vi "FlyWheelSim_Example.vi"() -> ()   [LabVIEW 2019]
uses:
  <vilib>/Rock Robotics/WPI/ThirdParty/JAS_Junk/TrajLib/TypeDef/DCMOTOR.CTL
  <vilib>/Rock Robotics/WPI/ThirdParty/JAS_Junk/TrajLib/TypeDef/LINEAR_SYSTEM.ctl
  <vilib>/Analysis/Matrix/Datatypes/RealMatrix.ctl
  <vilib>/Rock Robotics/WPI/ThirdParty/JAS_Junk/TrajLib/TypeDef/LINEAR_QUADRATIC_REGULATOR.ctl
  <vilib>/Rock Robotics/WPI/ThirdParty/JAS_Junk/TrajLib/TypeDef/KALMAN_FILTER.ctl
  <vilib>/Rock Robotics/WPI/ThirdParty/JAS_Junk/TrajLib/TypeDef/LINEAR_SYSTEM_LOOP.ctl
  <vilib>/Rock Robotics/WPI/ThirdParty/JAS_Junk/TrajLib/TypeDef/LINEAR_PLANT_INV_FF.ctl
  <vilib>/Rock Robotics/WPI/ThirdParty/JAS_Junk/TrajLib/TypeDef/FLYWHEEL_SIM.ctl
  <vilib>/Rock Robotics/WPI/ThirdParty/JAS_Junk/TrajLib/TypeDef/LINEAR_SYSTEM_SIM.ctl
  <vilib>/Rock Robotics/WPI/ThirdParty/JAS_Junk/TrajLib/MatBuilder_Create.vi
  <vilib>/Rock Robotics/WPI/ThirdParty/JAS_Junk/TrajLib/LinearFilter_ResetToValue.vi
  <vilib>/Rock Robotics/WPI/ThirdParty/JAS_Junk/TrajLib/LinearFilter_Calculate.vi
  <vilib>/Rock Robotics/WPI/ThirdParty/JAS_Junk/TrajLib/LinearFilter_MovingAverage.vi
  <vilib>/Rock Robotics/WPI/ThirdParty/JAS_Junk/TrajLib/LinearFilter_LowPassBW1.vi
  <vilib>/Rock Robotics/WPI/ThirdParty/JAS_Junk/TrajLib/LinearFilter_LowPassBW2.vi
  <vilib>/Rock Robotics/WPI/ThirdParty/JAS_Junk/TrajLib/LinearFilter_HighPassBW1.vi
  <vilib>/Rock Robotics/WPI/ThirdParty/JAS_Junk/TrajLib/LinearFilter_HighPassBW2.vi
  <vilib>/Rock Robotics/WPI/ThirdParty/JAS_Junk/TrajLib/Trajectory_Library.lvlib
  <vilib>/Analysis/Matrix/NI_Matrix.lvlib
panel:
  in  "Tab Control":T1(tab)
  out "Motor Current":dbl format="%20.3f"
  out "Battery \nVoltage":dbl format="%20.3f"
  in  "Shoot ball":bool
  out "CO Chart":T2(graph)
  in  "Shooter On/Off":bool
  out "Encoer Speed\nRad/Sec":dbl(slide) scale=0.0..300.0
  out "Speed":dbl format="%20.3f"
  out "Kalman Filtered\nSpeed":dbl format="%20.3f"
  out "PV Chart":T3(graph)
  out "Error":bool
  out "Motor Volt Dmd (CO)":dbl format="%20.3f"
  out "shoot Start":bool
  out "Shoot Done":bool
  out "Shooter Motor":T4 {"Jr_KgM2" format="%13.5p"; "L_H" format="%13.5p"; "Kt_NMPerAmp" format="%13.5p"; "KvINV_RadPerSecPerVolt" format="%13.5p"; "R_Ohms" format="%13.5p"; "FreeSpeed_RadPerSec" format="%13.5p"; "FreeCurrent_Amps" format="%13.5p"; "StallCurrent_Amps" format="%13.5p"; "StallTorque_NM" format="%13.5p"; "nominalVoltage_Volts" format="%13.5p"}
  out "m_flywheelPlant":T5
  out "m_FlyWheelSim":T7 {"GearBox"."Jr_KgM2" format="%13.5p"; "GearBox"."L_H" format="%13.5p"; "GearBox"."Kt_NMPerAmp" format="%13.5p"; "GearBox"."KvINV_RadPerSecPerVolt" format="%13.5p"; "GearBox"."R_Ohms" format="%13.5p"; "GearBox"."FreeSpeed_RadPerSec" format="%13.5p"; "GearBox"."FreeCurrent_Amps" format="%13.5p"; "GearBox"."StallCurrent_Amps" format="%13.5p"; "GearBox"."StallTorque_NM" format="%13.5p"; "GearBox"."nominalVoltage_Volts" format="%13.5p"}
  out "Shooting A":T6
  out "Shooting B":T6
  out "KalmanFilter":T9
  out "Kalman Error":errorcluster
  out "LinearQuadraticRegulator":T10
  out "LQR Error":bool
  out "Linear System Loop":T11
  out "LinSysLoop_Error":bool
  # "<States,States>"
  # "<States,Inputs>"
  # "<Outputs,States>"
  # "<Outputs,Inputs>"
  # "<States, 1>"
  # "<Outputs, 1>"
  # "<Inputs, 1>"
  # "<Outputs, 1>"
  # "<States,States>"
  # "<States,Inputs>"
  # "<Outputs,States>"
  # "<Outputs,Inputs>"
  # "Steady State Gain  \n<States,Outputs>"
  # "State Estimate <Statess,1>"
  # "<States,States>"
  # "<States,Inputs>"
  # "<Outputs,States>"
  # "<Outputs,Inputs>"
  # "Ref State <States,1>"
  # "Comp and capped \noutput <Inputs,1>"
  # "Controller gain\n<Inputs,States>"
  # "<States,1>"
  # "<FUTURE --- CLAMP TYPE -- For now\nuse Normalize>"
  # "Steady State Gain  \n<States,Outputs>"
  # "State Estimate <Statess,1>"
  # "<States,States>"
  # "<States,Inputs>"
  # "<Outputs,States>"
  # "<Outputs,Inputs>"
  # "<States,1>"
  # "<Inputs,1>"
  # "<States,Inputs>"
  # "<States,States>"
  # "Ref State <States,1>"
  # "Comp and capped \noutput <Inputs,1>"
  # "Controller gain\n<Inputs,States>"
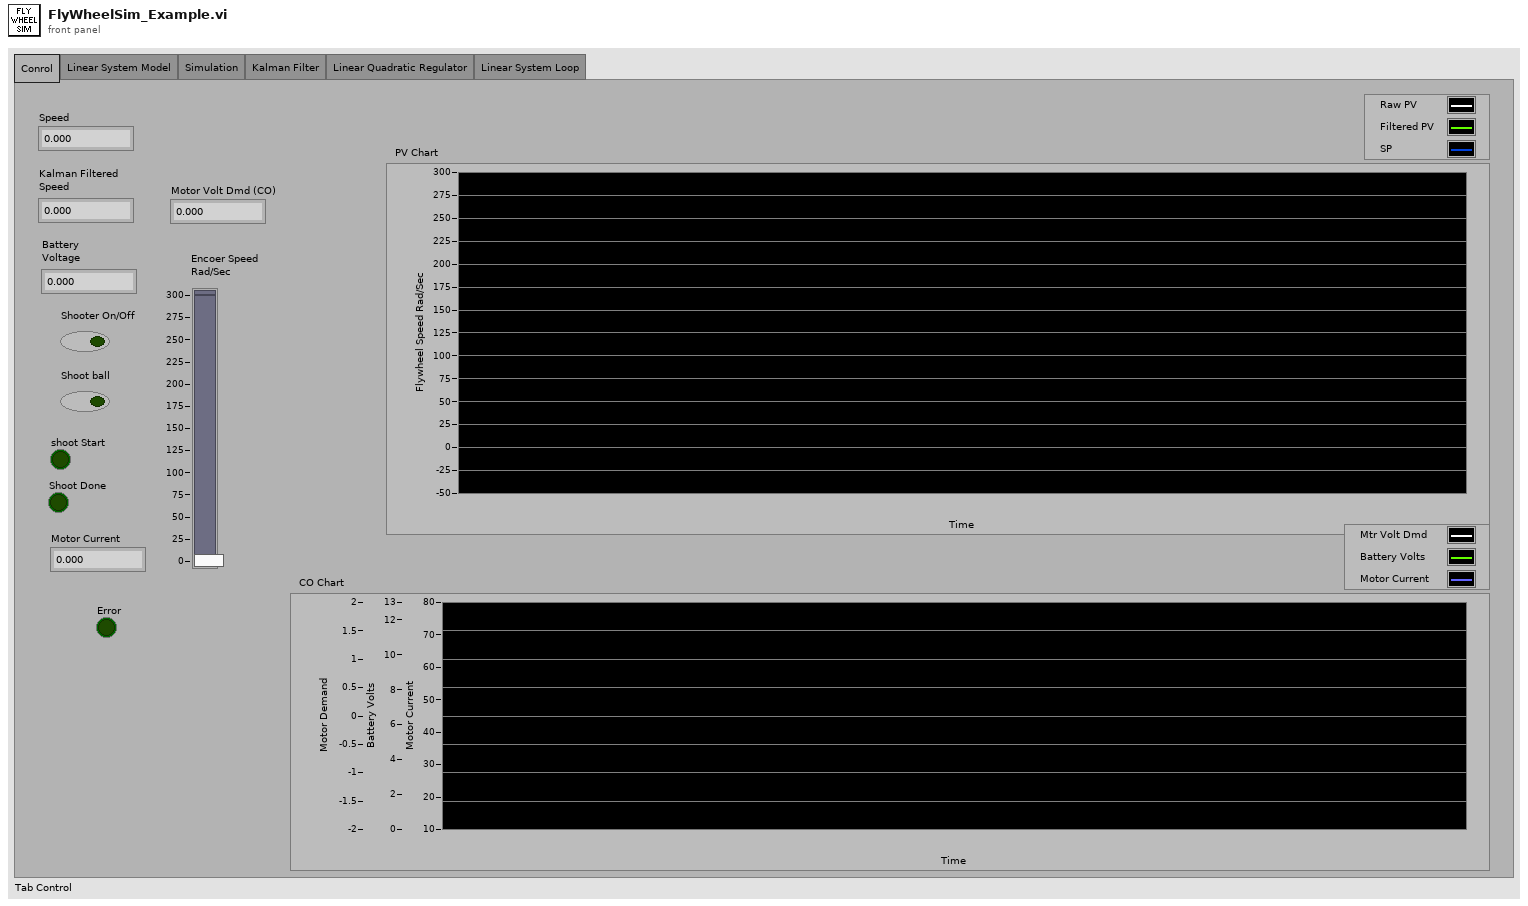
[diagram p1: front panel]
types:
  T1 = enum32{"Conrol", "Linear System Model", "Simulation", "Kalman Filter", "Linear Quadratic Regulator", "Linear System Loop"}
  T2 = cluster{"f":dbl, "Voltage":dbl, "Motor Current":dbl}
  T3 = cluster{"upper limit":dbl, "Real Matrix Element":dbl, "Real Matrix Element":dbl}
  T4 = typedef "Trajectory_Library.lvlib/DCMOTOR.CTL" = cluster{"nominalVoltage_Volts":dbl, "StallTorque_NM":dbl, "StallCurrent_Amps":dbl, "FreeCurrent_Amps":dbl, "FreeSpeed_RadPerSec":dbl, "R_Ohms":dbl, "KvINV_RadPerSecPerVolt":dbl, "Kt_NMPerAmp":dbl, "L_H":dbl, "Jr_KgM2":dbl}
  T5 = typedef "Trajectory_Library.lvlib/LINEAR_SYSTEM.ctl" = cluster{"m_A":T6, "m_B":T6, "m_C":T6, "m_D":T6, "States":i32, "Inputs":i32, "Outputs":i32}
  T6 = typedef "NI_Matrix.lvlib/RealMatrix.ctl" = dbl[][]
  T7 = typedef "Trajectory_Library.lvlib/FLYWHEEL_SIM.ctl" = cluster{"LinearSystemSim":T8, "GearBox":T4, "Gearing":dbl}
  T8 = typedef "Trajectory_Library.lvlib/LINEAR_SYSTEM_SIM.ctl" = cluster{"m_Plant":T5, "m_X":T6, "m_Y":T6, "m_U":T6, "MeasureStdDev":T6}
  T9 = typedef "Trajectory_Library.lvlib/KALMAN_FILTER.ctl" = cluster{"m_K":T6, "m_xHat":T6, "States":i32, "Outputs":i32, "m_Plant":T5}
  T10 = typedef "Trajectory_Library.lvlib/LINEAR_QUADRATIC_REGULATOR.ctl" = cluster{"m_r":T6, "m_U":T6, "m_K":T6, "States":i32, "Inputs":i32}
  T11 = typedef "Trajectory_Library.lvlib/LINEAR_SYSTEM_LOOP.ctl" = cluster{"Controller":T10, "FeedForward":T12, "Observer":T9, "Next_R":T6, "Clamp Max":T6}
  T12 = typedef "Trajectory_Library.lvlib/LINEAR_PLANT_INV_FF.ctl" = cluster{"m_R":T6, "m_Uff":T6, "m_B":T6, "m_A":T6, "States":i32, "Inputs":i32}
  T13 = enum16{"Moving Average", "Low Pass 1st Order Butterworth", "Low Pass 2nd Order Butterworth", "High Pass 1st Order Butterworth", "High Pass 2nd Order Butterworth"}
  T14 = cluster{"Velocity_RadPerSec":dbl, "Kalman FIltered\nVelocity (PV)":dbl, "Real Matrix Element":dbl}
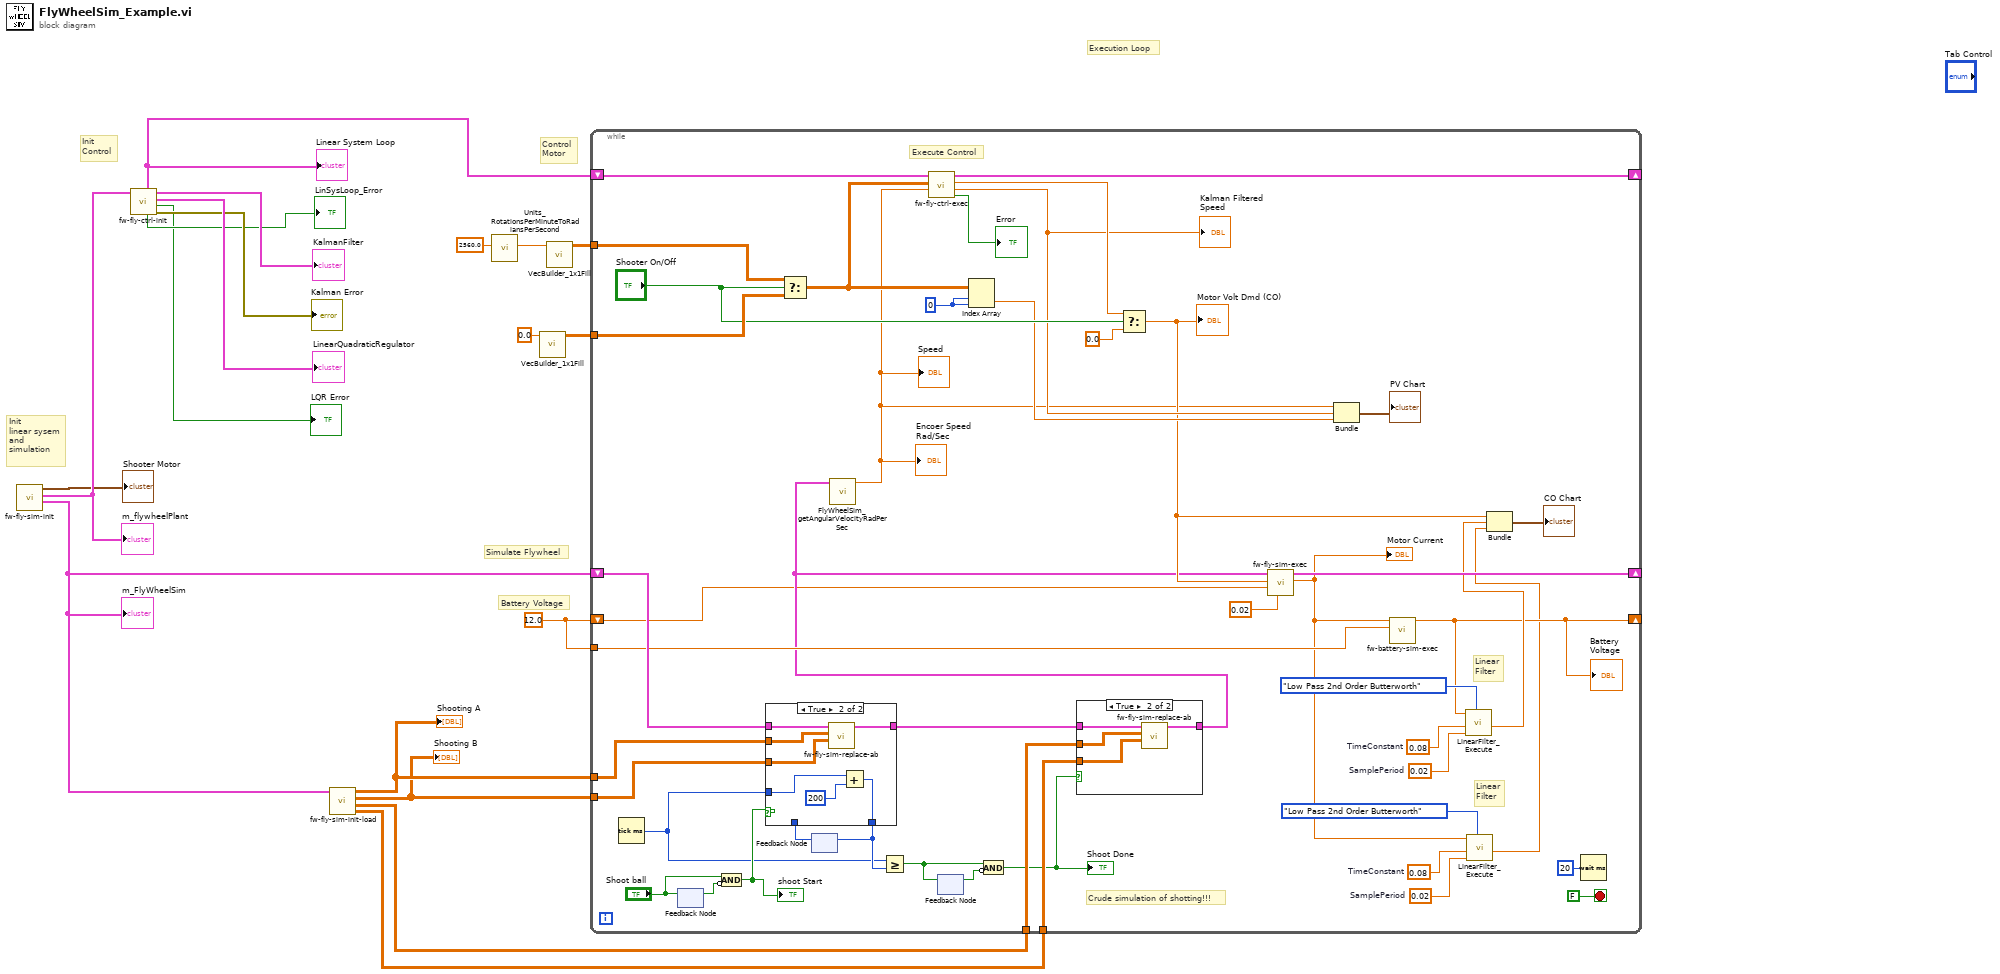
[diagram p0: block diagram]
diagram:
  w11 = 12.0
  # "Init\nlinear sysem\nand \nsimulation"
  # "Init\nControl"
  # "Execution Loop"
  # "Control\nMotor"
  # "Simulate Flywheel"
  # "Battery Voltage"
  n1 = call "fw-fly-sim-init.vi"() -> ("FlyWheelSim"=w10:T7, "Linearsystem"=w19:T5, "DCMOTOR"=→"Shooter Motor":T4)  [unwired: 9 in]
  "m_flywheelPlant" <- w19
  "m_FlyWheelSim" <- w10
  n2 = call "fw-fly-ctrl-init.vi"("Linearsystem"=w19) -> ("Kalman Error"=→"Kalman Error":errorcluster, "LQR Error"=→"LQR Error":bool, "LinearQuadraticRegulator"=→"LinearQuadraticRegulator":T10, "KalmanFilter"=→"KalmanFilter":T9, "Lin Sys Loop Error"=→"LinSysLoop_Error":bool, "Linear System Loop"=w1:T11)  [unwired: 5 in]
  "Linear System Loop" <- w1
  n3 = call "fw-fly-sim-init-load.vi"("FlyWheelSim"=w10) -> ("Normal B"=w5:T6, "Normal A"=w6:T6, "Loaded B"=w8:T6, "Loaded A"=w9:T6)  [unwired: 7 in]
  "Shooting A" <- w9
  "Shooting B" <- w8
  n4 = call <vilib>:"Units_RotationsPerMinuteToRadiansPerSecond.vi"("RotationsPerMinute"=2560.0) -> ("RadiansPerSecond"=w15:dbl)  [unwired: 10 in]
  n5 = call <vilib>:"VecBuilder_1x1Fill.vi"("R0_C0"=0.0) -> ("output matrix"=w12:T6)  [unwired: 10 in]
  n6 = call <vilib>:"VecBuilder_1x1Fill.vi"("R0_C0"=w15) -> ("output matrix"=w13:T6)  [unwired: 10 in]
  n7 = while {
    shift-right: [w64] -> _
    shift-left: w1 -> [w39]
    tunnel: w13 -> [w42]
    tunnel: w12 -> [w41]
    shift-right: [w62] -> _
    shift-left: w10 -> [w60]
    shift-right: [w22] -> _
    shift-left: w11 -> [w31]
    tunnel: w11 -> [w46]
    tunnel: w6 -> [w55]
    tunnel: w5 -> [w54]
    tunnel: w9 -> [w53]
    tunnel: w8 -> [w52]
    stop <- FALSE stop-if-true
    w26 = 0.02  # SamplePeriod
    w25 = 0.08  # TimeConstant
    w29 = 0.02  # SamplePeriod
    w28 = 0.08  # TimeConstant
    w63 = 0 ("index (row)")
    # "Linear\nFilter"
    # "Linear\nFilter"
    # "Execute Control"
    # "Crude simulation of shotting!!!"
    n8 = Tick Count (ms)() -> (millisecond timer value=w43:u32)
    n9 = feedback-in #1("Shoot ball") -> ()
    n10 = feedback #1() -> (w57:bool)  [unwired: 1 in]
    n11 = Compound Arithmetic op=AND("Shoot ball", invert w57) -> (w56:bool)
    "shoot Start" <- w56
    n12 = Select(t=w42, s="Shooter On/Off", f=w41) -> (s? t:f=w38:T6)
    n13 = feedback #2() -> (w47:u32)  [unwired: 1 in]
    n14 = case shown="True" w56 {
      tunnel: w60 -> [w74 w79]
      tunnel: [w74 w78] -> w59
      tunnel: w53 -> [_ w77]
      tunnel: w52 -> [_ w76]
      tunnel: [w73 w80] -> w48
      tunnel: w47 -> [w73 _]
      tunnel: w43 -> [_ w75]
      frame False {
      }
      frame True {
        n15 = call "fw-fly-sim-replace-ab.vi"("B"=w76, "A"=w77, "in FlyWheelSim"=w79) -> ("out FlyWheelSim"=w78:T7)  [unwired: 8 in]
        n16 = Add(x=w75, y=u32 200) -> (x+y=w80:u32)
      }
    }
    n17 = feedback-in #2(w48) -> ()
    n18 = Greater Or Equal?(x=w43, y=w48) -> (x >= y?=w50:bool)
    n19 = feedback #3() -> (w51:bool)  [unwired: 1 in]
    n20 = feedback-in #3(w50) -> ()
    n21 = Index Array(array=w38, index (row)=w63, index (col)=w63) -> (element=w35:dbl)
    n22 = Compound Arithmetic op=AND(w50, invert w51) -> (w49:bool)
    "Shoot Done" <- w49
    n23 = case shown="True" w49 {
      tunnel: w59 -> [w68 w72]
      tunnel: [w68 w71] -> w32
      tunnel: w55 -> [_ w70]
      tunnel: w54 -> [_ w69]
      frame False {
      }
      frame True {
        n24 = call "fw-fly-sim-replace-ab.vi"("B"=w69, "A"=w70, "in FlyWheelSim"=w72) -> ("out FlyWheelSim"=w71:T7)  [unwired: 8 in]
      }
    }
    n25 = call <vilib>:"FlyWheelSim_getAngularVelocityRadPerSec.vi"("FlyWheelSim"=w32) -> ("Velocity_RadPerSec"=w30:dbl)  [unwired: 10 in]
    "Encoer Speed\nRad/Sec" <- w30
    "Speed" <- w30
    n26 = call "fw-fly-ctrl-exec.vi"("Velocity (Rad/Sec)\n(PV)"=w30, "Velocity (Rad/Sec)\nSetpoint (SP)"=w38, "in Linear System Loop"=w39) -> ("Error"=→"Error":bool, "Kalman FIltered\nVelocity (PV)"=w37:dbl, "Motor Dmd"=w45:dbl, "out Linear System Loop"=w64:T11)  [unwired: 5 in]
    "Kalman Filtered\nSpeed" <- w37
    n27 = Select(t=w45, s="Shooter On/Off", f=0.0) -> (s? t:f=w33:dbl)
    "Motor Volt Dmd (CO)" <- w33
    n28 = call "fw-fly-sim-exec.vi"("dT_Seconds"=0.02, "Battery Voltage"=w31, "Motor Dmd (CO)"=w33, "in FlyWheelSim"=w32) -> ("Motor Current"=w21:dbl, "out FlyWheelSim"=w62:T7)  [unwired: 6 in]
    "Motor Current" <- w21
    n29 = Bundle("Velocity_RadPerSec"=w30, "Kalman FIltered\nVelocity (PV)"=w37, "Real Matrix Element"=w35) -> (→"PV Chart":T14)  [unwired: 1 in]
    n30 = call "fw-battery-sim-exec.vi"("Numeric"=w46, "Motor Current"=w21) -> ("Voltage"=w22:dbl)  [unwired: 9 in]
    "Battery \nVoltage" <- w22
    n31 = call <vilib>:"LinearFilter_Execute.vi"("Filter Type"=T13."Low Pass 2nd Order Butterworth", "SamplePeriod"=w29, "TimeConstant"=w28, "Input"=w22) -> ("Output"=w23:dbl)  [unwired: 6 in, 1 out]
    n32 = call <vilib>:"LinearFilter_Execute.vi"("Filter Type"=T13."Low Pass 2nd Order Butterworth", "SamplePeriod"=w26, "TimeConstant"=w25, "Input"=w21) -> ("Output"=w20:dbl)  [unwired: 6 in, 1 out]
    n33 = Bundle("f"=w33, "Output"=w23, "Output"=w20) -> (→"CO Chart":cluster{"f":dbl, "Output":dbl, "Output":dbl})  [unwired: 1 in]
    n34 = Wait (ms)(milliseconds to wait=u32 20) -> ()  [unwired: 1 out]
  }
